vi "from string.vi"(8 "error in":errorcluster, 9 "data":string, 10 "version":string, 11 "Daqmx Module configuration in":refnum<class "Daqmx Module configuration.lvclass">) -> (0 "error out":errorcluster, 3 "Daqmx Module configuration out":refnum<class "Daqmx Module configuration.lvclass">)   [LabVIEW 2015, in "DAQmx Module Configuration.lvclass"]
doc: "Provides an interface for loading a module configuration from a file or other serialized data source. It is recommended that all children of this class store data in two sets--data required for its own initialization, and any data required for parent initialization--and that each implementation uses the <b>Call Parent Method</b> primitive to de-serialize parent information. As a result, it is expected that every module configuration class calls <b>component configuration.lvclass:From String.vi</b>."
uses:
  Daqmx Module configuration.lvclass
  Line.ctl
  <vilib>/NI/Tag Bus Module Framework/channel/TBM channel.lvclass
  Measurement Type.ctl
  Parameters.ctl
  Daqmx Module Configuration 1_0_0 Typedef.ctl
  Daqmx Module configuration.lvclass/Daqmx Module configuration.ctl
  <vilib>/NI/Tag Bus Module Framework/module configuration/TBM module configuration.lvclass
  <vilib>/NI/Configuration Framework/serializable configuration/NISE_CEF_serializable configuration.lvclass
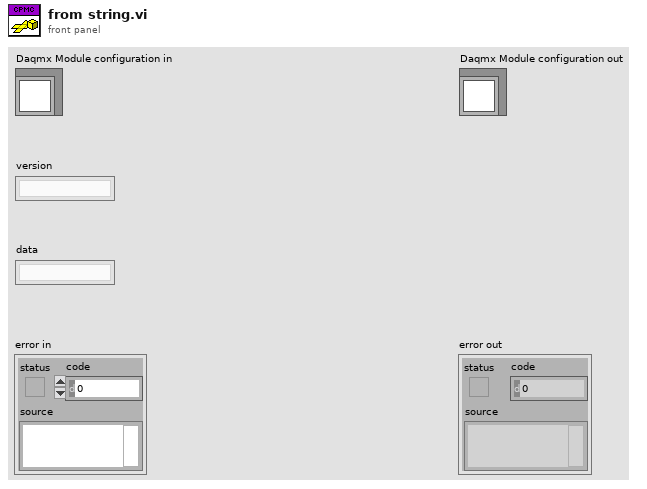
[diagram p1: front panel]
types:
  T1 = typedef "Daqmx Module configuration.lvclass/Daqmx Module Configuration 1_0_0 Typedef.ctl" = cluster{"channel":refnum<class "TBM channel.lvclass">, "Physical Channel":string, "Measurement Type":T2, "Parameters":cluster{"Digital Config":cluster{"Invert Lines?":bool}, "Voltage Config":cluster{"Maximum Value (V)":dbl, "Minimum Value (V)":dbl, "in terminal configuration (V)":i32, "out terminal configuration (V)":i32}, "Current Config":cluster{"Maximum Value (A)":dbl, "Minimum Value (A)":dbl, "shunt resistor location":i32, "input terminal configuration (C)":i32, "external shunt resistor value":dbl}, "RTD Config":cluster{"Maximum Value (°C)":dbl, "Minimum Value (°C)":dbl, "resistance configuration":i32, "r0":dbl, "current excitation value":dbl, "rtd type":i32, "current excitation source":i32}, "Thermocouple Config":cluster{"Minimum Value (C)":dbl, "Maximum Value (C)":dbl, "thermocouple type":i32, "cjc source":i32, "cjc value":dbl}, "Strain Config":cluster{"Maximum Value":dbl, "Minimum Value":dbl, "bridge information":cluster{"strain configuration":i32, "lead wire resistance":dbl, "initial bridge voltage":dbl, "voltage excitation source":i32, "voltage excitation value":dbl}, "strain gage information":cluster{"gage factor":dbl, "nominal gage resistance":dbl, "poisson ratio":dbl}}}}
  T2 = typedef "DAQmx Module Configuration.lvclass/Measurement Type.ctl" = enum16{"Digital Input", "Digital Output", "Voltage Input", "Voltage Output", "Current Input", "Current Output", "RTD", "Thermocouple", "Strain", "PWM"}
  T3 = typedef "DAQmx Module Configuration.lvclass/Line.ctl" = cluster{"Channel Array":refnum<class "TBM channel.lvclass">[], "Physical Channel":string, "Measurement Type":T2, "Parameters":T4}
  T4 = typedef "DAQmx Module Configuration.lvclass/Parameters.ctl" = cluster{"Digital Config":cluster{"Invert Lines?":bool}, "Voltage Config":cluster{"Maximum Value (V)":dbl, "Minimum Value (V)":dbl, "in terminal configuration (V)":i32, "out terminal configuration (V)":i32}, "Current Config":cluster{"Maximum Value (A)":dbl, "Minimum Value (A)":dbl, "shunt resistor location":i32, "input terminal configuration (C)":i32, "external shunt resistor value":dbl}, "RTD Config":cluster{"Maximum Value (°C)":dbl, "Minimum Value (°C)":dbl, "resistance configuration":i32, "r0":dbl, "current excitation value":dbl, "rtd type":i32, "current excitation source":i32}, "Thermocouple Config":cluster{"Minimum Value (C)":dbl, "Maximum Value (C)":dbl, "thermocouple type":i32, "cjc source":i32, "cjc value":dbl}, "Strain Config":cluster{"Maximum Value":dbl, "Minimum Value":dbl, "bridge information":cluster{"strain configuration":i32, "lead wire resistance":dbl, "initial bridge voltage":dbl, "voltage excitation source":i32, "voltage excitation value":dbl}, "strain gage information":cluster{"gage factor":dbl, "nominal gage resistance":dbl, "poisson ratio":dbl}}, "PWM Config":cluster{"Idle State":bool}}
  T5 = cluster{"Digital Config":cluster{"Invert Lines?":bool}, "Voltage Config":cluster{"Maximum Value (V)":dbl, "Minimum Value (V)":dbl, "in terminal configuration (V)":i32, "out terminal configuration (V)":i32}, "Current Config":cluster{"Maximum Value (A)":dbl, "Minimum Value (A)":dbl, "shunt resistor location":i32, "input terminal configuration (C)":i32, "external shunt resistor value":dbl}, "RTD Config":cluster{"Maximum Value (°C)":dbl, "Minimum Value (°C)":dbl, "resistance configuration":i32, "r0":dbl, "current excitation value":dbl, "rtd type":i32, "current excitation source":i32}, "Thermocouple Config":cluster{"Minimum Value (C)":dbl, "Maximum Value (C)":dbl, "thermocouple type":i32, "cjc source":i32, "cjc value":dbl}, "Strain Config":cluster{"Maximum Value":dbl, "Minimum Value":dbl, "bridge information":cluster{"strain configuration":i32, "lead wire resistance":dbl, "initial bridge voltage":dbl, "voltage excitation source":i32, "voltage excitation value":dbl}, "strain gage information":cluster{"gage factor":dbl, "nominal gage resistance":dbl, "poisson ratio":dbl}}}
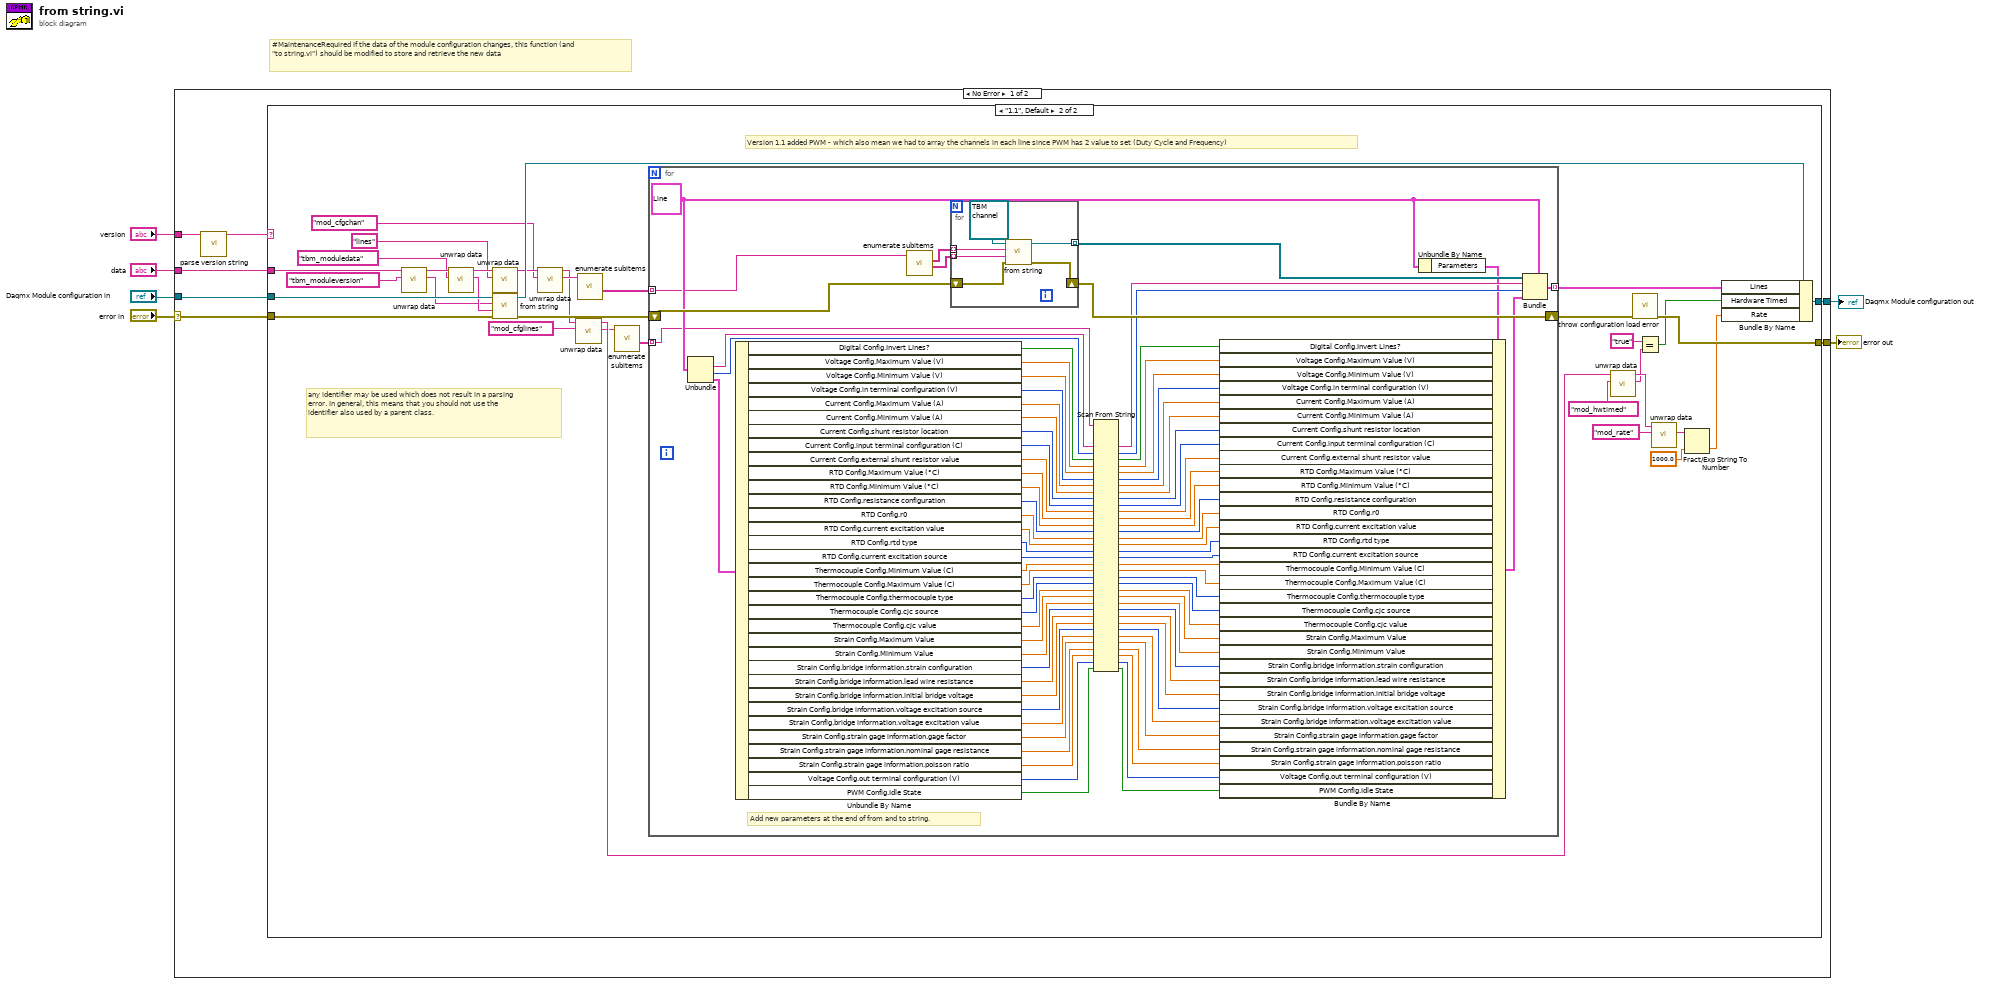
[diagram p0: block diagram]
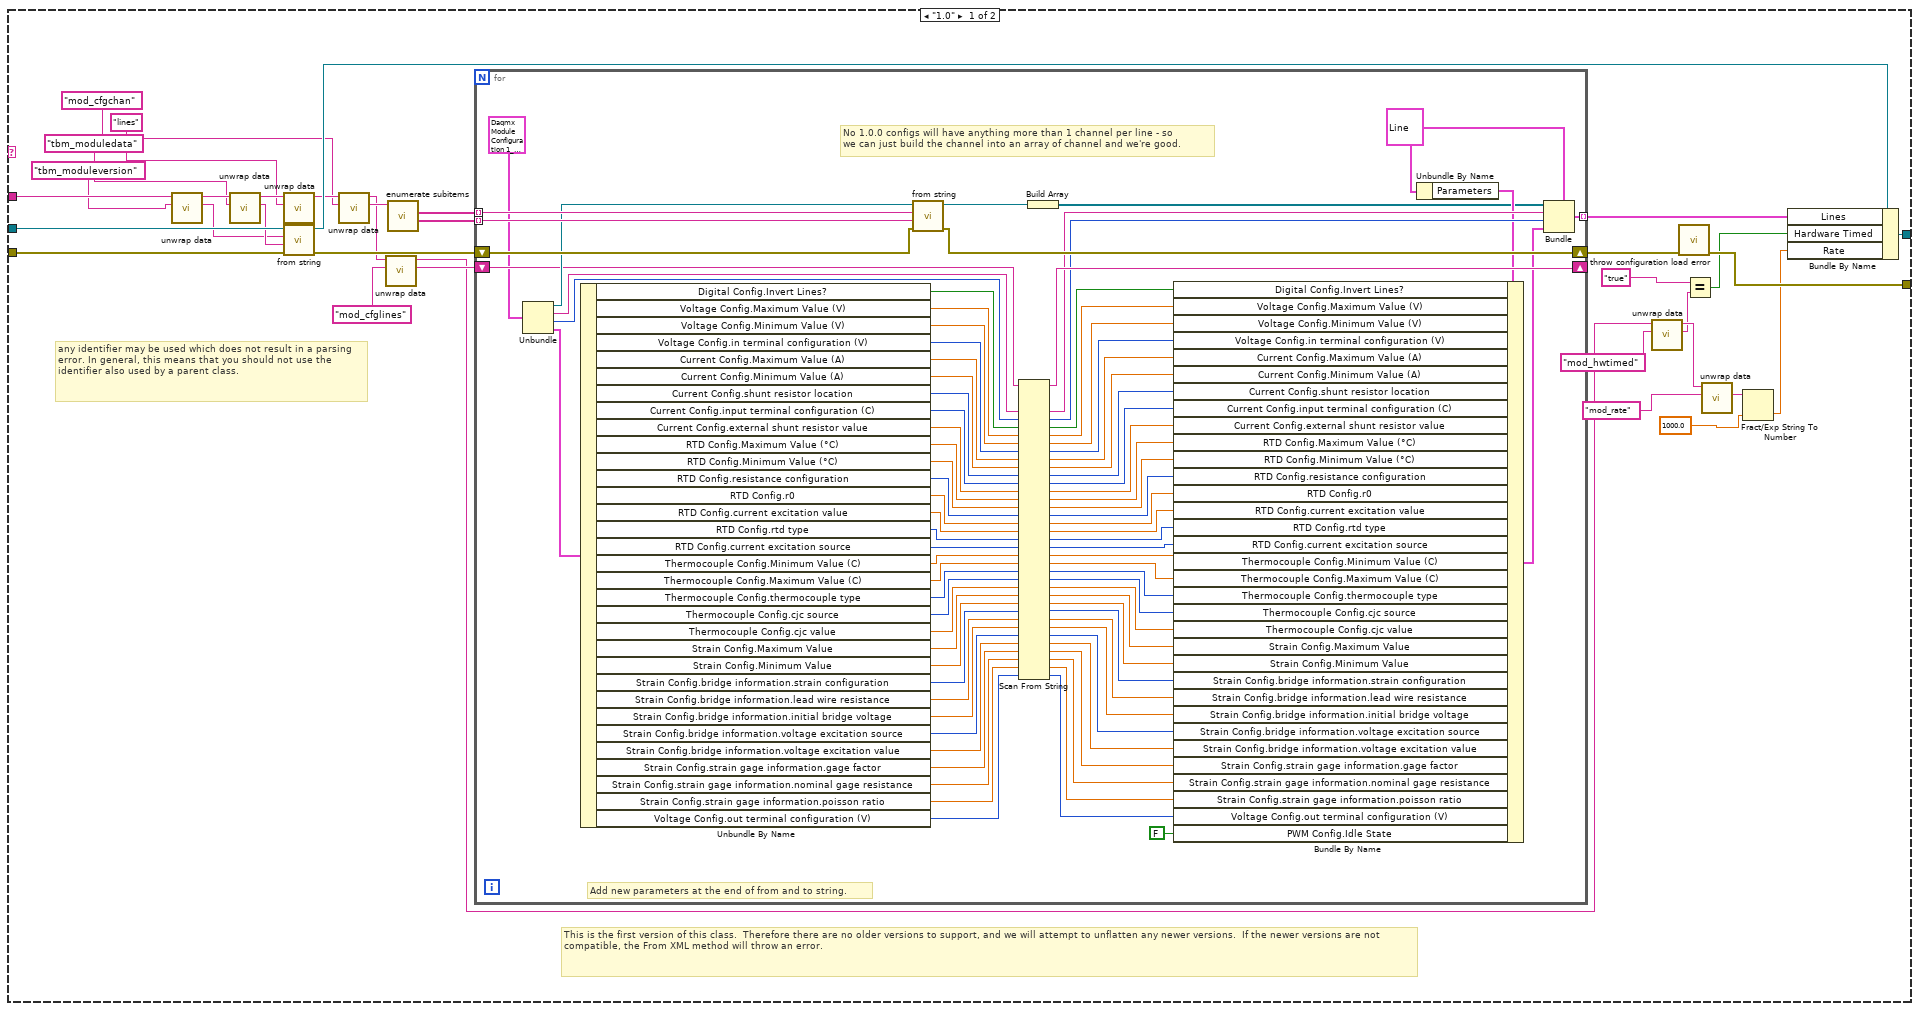
[diagram p2: hidden frame]
diagram:
  # "#MaintenanceRequired If the data of the module configuration changes, this function (and \"to string.vi\") should be modified to store and retrieve the new data"
  n1 = case shown="No Error" "error in" {
    selector: "error in" -> [w7 w255]
    tunnel: "data" -> [w13 _]
    tunnel: "Daqmx Module configuration in" -> [w12 w254]
    tunnel: [w11 w254] -> w1
    tunnel: [w10 w255] -> w6
    tunnel: "version" -> [w9 _]
    frame No Error {
      n2 = call <vilib>:"parse version string.vi"("full version"=w9) -> ("major.minor version"=w8:string)  [unwired: 7 in, 3 out]
      n3 = case shown="\"1.1\", Default" w8 {
        tunnel: w13 -> [w44 w162]
        tunnel: w7 -> [w43 w161]
        tunnel: w12 -> [w47 w165]
        tunnel: [w35 w153] -> w11
        tunnel: [w46 w164] -> w10
        frame "1.0" {
          # "This is the first version of this class.  Therefore there are no older versions to support, and we will attempt to unflatten any newer versions.  If the newer versions are not compatible, the From XML method will throw an error."
          # "any identifier may be used which does not result in a parsing error. In general, this means that you should not use the identifier also used by a parent class."
          n4 = call <vilib>:"unwrap data.vi"("identifier"="tbm_moduleversion" ("additional identifier"), "data to unwrap"=w44) -> ("unwrapped data"=w39:string, "remaining string"=w45:string)  [unwired: 8 in]
          n5 = call <vilib>:"unwrap data.vi"("identifier"="tbm_moduledata" ("additional identifier"), "data to unwrap"=w45) -> ("unwrapped data"=w41:string, "remaining string"=w38:string)  [unwired: 8 in]
          n6 = call <vilib>:"unwrap data.vi"("identifier"="lines" ("additional identifier"), "data to unwrap"=w38) -> ("remaining string"=w34:string)  [unwired: 8 in, 1 out]
          n7 = call-parent "from string.vi"("error in"=w43, "data"=w41, "version"=w39, "module configuration in"=w47) -> ("error out"=w30:errorcluster, "module configuration out"=w36:refnum<class "Daqmx Module configuration.lvclass">)  [unwired: 6 in]
          n8 = call <vilib>:"unwrap data.vi"("identifier"="mod_cfgchan", "data to unwrap"=w34) -> ("unwrapped data"=w29:string, "remaining string"=w26:string)  [unwired: 8 in]
          n9 = call <vilib>:"unwrap data.vi"("identifier"="mod_cfglines", "data to unwrap"=w26) -> ("unwrapped data"=w24:string, "remaining string"=w14:string)  [unwired: 8 in]
          n10 = call <vilib>:"enumerate subitems.vi"("data to enumerate"=w29) -> ("associated data"=w31:string[], "discovered subitems"=w32:string[])  [unwired: 8 in, 1 out]
          n11 = for {
            shift-right: [w126] -> w28
            shift-left: w30 -> [w131]
            tunnel: w32 -> [w130] mode=indexing
            tunnel: w31 -> [w129] mode=indexing
            tunnel: [w127] -> w27 mode=indexing
            shift-right: [w98] -> _
            shift-left: w24 -> [w99]
            w54 = T3 {"Channel Array"=[], "Physical Channel"="", "Measurement Type"=enum."Digital Input", "Parameters"={"Digital Config"={"Invert Lines?"=FALSE}, "Voltage Config"={"Maximum Value (V)"=5.0, "Minimum Value (V)"=-5.0, "in terminal configuration (V)"=-1, "out terminal configuration (V)"=-1}, "Current Config"={"Maximum Value (A)"=0.02, "Minimum Value (A)"=0.0, "shunt resistor location"=-1, "input terminal configuration (C)"=-1, "external shunt resistor value"=249.0}, "RTD Config"={"Maximum Value (°C)"=100.0, "Minimum Value (°C)"=0.0, "resistance configuration"=2, "r0"=100.0, "current excitation value"=0.0025, "rtd type"=10137, "current excitation source"=10167}, "Thermocouple Config"={"Minimum Value (C)"=0.0, "Maximum Value (C)"=100.0, "thermocouple type"=10072, "cjc source"=10116, "cjc value"=25.0}, "Strain Config"={"Maximum Value"=0.001, "Minimum Value"=-0.001, "bridge information"={"strain configuration"=10183, "lead wire resistance"=0.0, "initial bridge voltage"=0.0, "voltage excitation source"=10200, "voltage excitation value"=2.5}, "strain gage information"={"gage factor"=2.0, "nominal gage resistance"=350.0, "poisson ratio"=0.3}}, "PWM Config"={"Idle State"=FALSE}}} ("Line")
            # "No 1.0.0 configs will have anything more than 1 channel per line - so\nwe can just build the channel into an array of channel and we're good."
            # "Add new parameters at the end of from and to string."
            n12 = Unbundle(T1 {"channel"=refnum, "Physical Channel"="", "Measurement Type"=enum."Digital Input", "Parameters"={"Digital Config"={"Invert Lines?"=FALSE}, "Voltage Config"={"Maximum Value (V)"=5.0, "Minimum Value (V)"=-5.0, "in terminal configuration (V)"=-1, "out terminal configuration (V)"=-1}, "Current Config"={"Maximum Value (A)"=0.02, "Minimum Value (A)"=0.0, "shunt resistor location"=-1, "input terminal configuration (C)"=-1, "external shunt resistor value"=249.0}, "RTD Config"={"Maximum Value (°C)"=100.0, "Minimum Value (°C)"=0.0, "resistance configuration"=2, "r0"=100.0, "current excitation value"=0.0025, "rtd type"=10137, "current excitation source"=10167}, "Thermocouple Config"={"Minimum Value (C)"=0.0, "Maximum Value (C)"=100.0, "thermocouple type"=10072, "cjc source"=10116, "cjc value"=25.0}, "Strain Config"={"Maximum Value"=0.001, "Minimum Value"=-0.001, "bridge information"={"strain configuration"=10183, "lead wire resistance"=0.0, "initial bridge voltage"=0.0, "voltage excitation source"=10200, "voltage excitation value"=2.5}, "strain gage information"={"gage factor"=2.0, "nominal gage resistance"=350.0, "poisson ratio"=0.3}}}} ("1.0 Config")) -> ("channel"=w125:refnum<class "TBM channel.lvclass">, "Physical Channel"=w124:string, "Measurement Type"=w100:T2, "Parameters"=w96:T5)
            n13 = Unbundle By Name(w96) -> ("Digital Config.Invert Lines?"=w123:bool, "Voltage Config.Maximum Value (V)"=w122:dbl, "Voltage Config.Minimum Value (V)"=w121:dbl, "Voltage Config.in terminal configuration (V)"=w120:i32, "Current Config.Maximum Value (A)"=w119:dbl, "Current Config.Minimum Value (A)"=w118:dbl, "Current Config.shunt resistor location"=w117:i32, "Current Config.input terminal configuration (C)"=w116:i32, "Current Config.external shunt resistor value"=w114:dbl, "RTD Config.Maximum Value (°C)"=w115:dbl, "RTD Config.Minimum Value (°C)"=w113:dbl, "RTD Config.resistance configuration"=w112:i32, "RTD Config.r0"=w111:dbl, "RTD Config.current excitation value"=w110:dbl, "RTD Config.rtd type"=w109:i32, "RTD Config.current excitation source"=w108:i32, "Thermocouple Config.Minimum Value (C)"=w107:dbl, "Thermocouple Config.Maximum Value (C)"=w106:dbl, "Thermocouple Config.thermocouple type"=w105:i32, "Thermocouple Config.cjc source"=w104:i32, "Thermocouple Config.cjc value"=w103:dbl, "Strain Config.Maximum Value"=w102:dbl, "Strain Config.Minimum Value"=w101:dbl, "Strain Config.bridge information.strain configuration"=w95:i32, "Strain Config.bridge information.lead wire resistance"=w94:dbl, "Strain Config.bridge information.initial bridge voltage"=w93:dbl, "Strain Config.bridge information.voltage excitation source"=w92:i32, "Strain Config.bridge information.voltage excitation value"=w91:dbl, "Strain Config.strain gage information.gage factor"=w90:dbl, "Strain Config.strain gage information.nominal gage resistance"=w89:dbl, "Strain Config.strain gage information.poisson ratio"=w88:dbl, "Voltage Config.out terminal configuration (V)"=w52:i32)
            n14 = call-dynamic "from string.vi"("error in"=w131, "channel data"=w129, "identifier"=w130, "channel in"=w125) -> ("error out"=w126:errorcluster, "channel out"=w128:refnum<class "TBM channel.lvclass">)  [unwired: 6 in]
            n15 = Scan From String(input string=w99, default 1=w124, default 2=w100, default 3=w123, default 4=w122, default 5=w121, default 6=w120, default 7=w119, default 8=w118, default 9=w117, default 10=w116, default 11=w114, default 12=w115, default 13=w113, default 14=w112, default 15=w111, default 16=w110, default 17=w109, default 18=w108, default 19=w107, default 20=w106, default 21=w105, default 22=w104, default 23=w103, default 24=w102, default 25=w101, default 26=w95, default 27=w94, default 28=w93, default 29=w92, default 30=w91, default 31=w90, default 32=w89, default 33=w88, default 34=w52) -> (remaining string=w98:string, output 1=w97:string, output 2=w87:T2, output 3=w86:bool, output 4=w85:dbl, output 5=w84:dbl, output 6=w83:i32, output 7=w82:dbl, output 8=w81:dbl, output 9=w80:i32, output 10=w79:i32, output 11=w78:dbl, output 12=w77:dbl, output 13=w76:dbl, output 14=w75:i32, output 15=w74:dbl, output 16=w73:dbl, output 17=w72:i32, output 18=w71:i32, output 19=w70:dbl, output 20=w69:dbl, output 21=w68:i32, output 22=w67:i32, output 23=w66:dbl, output 24=w65:dbl, output 25=w64:dbl, output 26=w63:i32, output 27=w62:dbl, output 28=w61:dbl, output 29=w60:i32, output 30=w59:dbl, output 31=w58:dbl, output 32=w57:dbl, output 33=w56:dbl, output 34=w51:i32)  [unwired: 3 in, 2 out]
            n16 = Build Array(w128) -> (w50:refnum<class "TBM channel.lvclass">[])
            n17 = Unbundle By Name(w54) -> ("Parameters"=w53:T4)
            n18 = Bundle By Name(cluster=w53, "Digital Config.Invert Lines?"=w86, "Voltage Config.Maximum Value (V)"=w85, "Voltage Config.Minimum Value (V)"=w84, "Voltage Config.in terminal configuration (V)"=w83, "Current Config.Maximum Value (A)"=w82, "Current Config.Minimum Value (A)"=w81, "Current Config.shunt resistor location"=w80, "Current Config.input terminal configuration (C)"=w79, "Current Config.external shunt resistor value"=w78, "RTD Config.Maximum Value (°C)"=w77, "RTD Config.Minimum Value (°C)"=w76, "RTD Config.resistance configuration"=w75, "RTD Config.r0"=w74, "RTD Config.current excitation value"=w73, "RTD Config.rtd type"=w72, "RTD Config.current excitation source"=w71, "Thermocouple Config.Minimum Value (C)"=w70, "Thermocouple Config.Maximum Value (C)"=w69, "Thermocouple Config.thermocouple type"=w68, "Thermocouple Config.cjc source"=w67, "Thermocouple Config.cjc value"=w66, "Strain Config.Maximum Value"=w65, "Strain Config.Minimum Value"=w64, "Strain Config.bridge information.strain configuration"=w63, "Strain Config.bridge information.lead wire resistance"=w62, "Strain Config.bridge information.initial bridge voltage"=w61, "Strain Config.bridge information.voltage excitation source"=w60, "Strain Config.bridge information.voltage excitation value"=w59, "Strain Config.strain gage information.gage factor"=w58, "Strain Config.strain gage information.nominal gage resistance"=w57, "Strain Config.strain gage information.poisson ratio"=w56, "Voltage Config.out terminal configuration (V)"=w51, "PWM Config.Idle State"=FALSE) -> (w55:T4)
            n19 = Bundle(cluster=w54, "Channel Array"=w50, "Physical Channel"=w97, "Measurement Type"=w87, "Parameters"=w55) -> (w127:T3)
          }
          n20 = call <vilib>:"unwrap data.vi"("identifier"="mod_hwtimed", "data to unwrap"=w14) -> ("unwrapped data"=w20:string, "remaining string"=w21:string)  [unwired: 8 in]
          n21 = call <vilib>:"throw configuration load error.vi"("error in"=w28) -> ("error out"=w46:errorcluster)  [unwired: 10 in]
          n22 = Equal?(x="true" ("identifier"), y=w20) -> (x = y?=w18:bool)
          n23 = call <vilib>:"unwrap data.vi"("identifier"="mod_rate", "data to unwrap"=w21) -> ("unwrapped data"=w17:string)  [unwired: 8 in, 1 out]
          n24 = Fract/Exp String To Number(string=w17, default (0 dbl)=1000.0 ("default (0 DBL)")) -> (number=w16:dbl)  [unwired: 2 in, 1 out]
          n25 = Bundle By Name(cluster=w36, "Lines"=w27, "Hardware Timed"=w18, "Rate"=w16) -> (w35:refnum<class "Daqmx Module configuration.lvclass">)
        }
        frame "1.1", Default {
          # "Version 1.1 added PWM - which also mean we had to array the channels in each line since PWM has 2 value to set (Duty Cycle and Frequency)"
          # "any identifier may be used which does not result in a parsing error. In general, this means that you should not use the identifier also used by a parent class."
          n26 = call <vilib>:"unwrap data.vi"("identifier"="tbm_moduleversion" ("additional identifier"), "data to unwrap"=w162) -> ("unwrapped data"=w157:string, "remaining string"=w163:string)  [unwired: 8 in]
          n27 = call <vilib>:"unwrap data.vi"("identifier"="tbm_moduledata" ("additional identifier"), "data to unwrap"=w163) -> ("unwrapped data"=w159:string, "remaining string"=w156:string)  [unwired: 8 in]
          n28 = call <vilib>:"unwrap data.vi"("identifier"="lines" ("additional identifier"), "data to unwrap"=w156) -> ("remaining string"=w152:string)  [unwired: 8 in, 1 out]
          n29 = call-parent "from string.vi"("error in"=w161, "data"=w159, "version"=w157, "module configuration in"=w165) -> ("error out"=w149:errorcluster, "module configuration out"=w154:refnum<class "Daqmx Module configuration.lvclass">)  [unwired: 6 in]
          n30 = call <vilib>:"unwrap data.vi"("identifier"="mod_cfgchan", "data to unwrap"=w152) -> ("unwrapped data"=w148:string, "remaining string"=w145:string)  [unwired: 8 in]
          n31 = call <vilib>:"unwrap data.vi"("identifier"="mod_cfglines", "data to unwrap"=w145) -> ("unwrapped data"=w133:string, "remaining string"=w134:string)  [unwired: 8 in]
          n32 = call <vilib>:"enumerate subitems.vi"("data to enumerate"=w148) -> ("associated data"=w150:string[])  [unwired: 8 in, 2 out]
          n33 = call <vilib>:"enumerate subitems.vi"("data to enumerate"=w133) -> ("associated data"=w132:string[])  [unwired: 8 in, 2 out]
          n34 = for {
            shift-right: [w244] -> w147
            shift-left: w149 -> [w247]
            tunnel: w150 -> [w167] mode=indexing
            tunnel: [w245] -> w146 mode=indexing
            tunnel: w132 -> [w166] mode=indexing
            w175 = T3 {"Channel Array"=[], "Physical Channel"="", "Measurement Type"=enum."Digital Input", "Parameters"={"Digital Config"={"Invert Lines?"=FALSE}, "Voltage Config"={"Maximum Value (V)"=5.0, "Minimum Value (V)"=-5.0, "in terminal configuration (V)"=-1, "out terminal configuration (V)"=-1}, "Current Config"={"Maximum Value (A)"=0.02, "Minimum Value (A)"=0.0, "shunt resistor location"=-1, "input terminal configuration (C)"=-1, "external shunt resistor value"=249.0}, "RTD Config"={"Maximum Value (°C)"=100.0, "Minimum Value (°C)"=0.0, "resistance configuration"=2, "r0"=100.0, "current excitation value"=0.0025, "rtd type"=10137, "current excitation source"=10167}, "Thermocouple Config"={"Minimum Value (C)"=0.0, "Maximum Value (C)"=100.0, "thermocouple type"=10072, "cjc source"=10116, "cjc value"=25.0}, "Strain Config"={"Maximum Value"=0.001, "Minimum Value"=-0.001, "bridge information"={"strain configuration"=10183, "lead wire resistance"=0.0, "initial bridge voltage"=0.0, "voltage excitation source"=10200, "voltage excitation value"=2.5}, "strain gage information"={"gage factor"=2.0, "nominal gage resistance"=350.0, "poisson ratio"=0.3}}, "PWM Config"={"Idle State"=FALSE}}} ("Line")
            # "Add new parameters at the end of from and to string."
            n35 = Unbundle(w175) -> ("Physical Channel"=w243:string, "Measurement Type"=w219:T2, "Parameters"=w217:T4)  [unwired: 1 out]
            n36 = Unbundle By Name(w217) -> ("Digital Config.Invert Lines?"=w242:bool, "Voltage Config.Maximum Value (V)"=w241:dbl, "Voltage Config.Minimum Value (V)"=w240:dbl, "Voltage Config.in terminal configuration (V)"=w239:i32, "Current Config.Maximum Value (A)"=w238:dbl, "Current Config.Minimum Value (A)"=w237:dbl, "Current Config.shunt resistor location"=w236:i32, "Current Config.input terminal configuration (C)"=w235:i32, "Current Config.external shunt resistor value"=w233:dbl, "RTD Config.Maximum Value (°C)"=w234:dbl, "RTD Config.Minimum Value (°C)"=w232:dbl, "RTD Config.resistance configuration"=w231:i32, "RTD Config.r0"=w230:dbl, "RTD Config.current excitation value"=w229:dbl, "RTD Config.rtd type"=w228:i32, "RTD Config.current excitation source"=w227:i32, "Thermocouple Config.Minimum Value (C)"=w226:dbl, "Thermocouple Config.Maximum Value (C)"=w225:dbl, "Thermocouple Config.thermocouple type"=w224:i32, "Thermocouple Config.cjc source"=w223:i32, "Thermocouple Config.cjc value"=w222:dbl, "Strain Config.Maximum Value"=w221:dbl, "Strain Config.Minimum Value"=w220:dbl, "Strain Config.bridge information.strain configuration"=w216:i32, "Strain Config.bridge information.lead wire resistance"=w215:dbl, "Strain Config.bridge information.initial bridge voltage"=w214:dbl, "Strain Config.bridge information.voltage excitation source"=w213:i32, "Strain Config.bridge information.voltage excitation value"=w212:dbl, "Strain Config.strain gage information.gage factor"=w211:dbl, "Strain Config.strain gage information.nominal gage resistance"=w210:dbl, "Strain Config.strain gage information.poisson ratio"=w209:dbl, "Voltage Config.out terminal configuration (V)"=w173:i32, "PWM Config.Idle State"=w171:bool)
            n37 = call <vilib>:"enumerate subitems.vi"("data to enumerate"=w167) -> ("associated data"=w168:string[], "discovered subitems"=w169:string[])  [unwired: 8 in, 1 out]
            n38 = for {
              tunnel: w169 -> [w250] mode=indexing
              tunnel: w168 -> [w249] mode=indexing
              tunnel: [w252] -> w246 mode=indexing
              shift-right: [w251] -> w244
              shift-left: w247 -> [w253]
              n39 = call-dynamic "from string.vi"("error in"=w253, "channel data"=w249, "identifier"=w250, "channel in"=refnum<class "TBM channel.lvclass"> refnum) -> ("error out"=w251:errorcluster, "channel out"=w252:refnum<class "TBM channel.lvclass">)  [unwired: 6 in]
            }
            n40 = Scan From String(input string=w166, default 1=w243, default 2=w219, default 3=w242, default 4=w241, default 5=w240, default 6=w239, default 7=w238, default 8=w237, default 9=w236, default 10=w235, default 11=w233, default 12=w234, default 13=w232, default 14=w231, default 15=w230, default 16=w229, default 17=w228, default 18=w227, default 19=w226, default 20=w225, default 21=w224, default 22=w223, default 23=w222, default 24=w221, default 25=w220, default 26=w216, default 27=w215, default 28=w214, default 29=w213, default 30=w212, default 31=w211, default 32=w210, default 33=w209, default 34=w173, default 35=w171) -> (output 1=w218:string, output 2=w208:T2, output 3=w207:bool, output 4=w206:dbl, output 5=w205:dbl, output 6=w204:i32, output 7=w203:dbl, output 8=w202:dbl, output 9=w201:i32, output 10=w200:i32, output 11=w199:dbl, output 12=w198:dbl, output 13=w197:dbl, output 14=w196:i32, output 15=w195:dbl, output 16=w194:dbl, output 17=w193:i32, output 18=w192:i32, output 19=w191:dbl, output 20=w190:dbl, output 21=w189:i32, output 22=w188:i32, output 23=w187:dbl, output 24=w186:dbl, output 25=w185:dbl, output 26=w184:i32, output 27=w183:dbl, output 28=w182:dbl, output 29=w181:i32, output 30=w180:dbl, output 31=w179:dbl, output 32=w178:dbl, output 33=w177:dbl, output 34=w172:i32, output 35=w170:bool)  [unwired: 3 in, 3 out]
            n41 = Unbundle By Name(w175) -> ("Parameters"=w174:T4)
            n42 = Bundle By Name(cluster=w174, "Digital Config.Invert Lines?"=w207, "Voltage Config.Maximum Value (V)"=w206, "Voltage Config.Minimum Value (V)"=w205, "Voltage Config.in terminal configuration (V)"=w204, "Current Config.Maximum Value (A)"=w203, "Current Config.Minimum Value (A)"=w202, "Current Config.shunt resistor location"=w201, "Current Config.input terminal configuration (C)"=w200, "Current Config.external shunt resistor value"=w199, "RTD Config.Maximum Value (°C)"=w198, "RTD Config.Minimum Value (°C)"=w197, "RTD Config.resistance configuration"=w196, "RTD Config.r0"=w195, "RTD Config.current excitation value"=w194, "RTD Config.rtd type"=w193, "RTD Config.current excitation source"=w192, "Thermocouple Config.Minimum Value (C)"=w191, "Thermocouple Config.Maximum Value (C)"=w190, "Thermocouple Config.thermocouple type"=w189, "Thermocouple Config.cjc source"=w188, "Thermocouple Config.cjc value"=w187, "Strain Config.Maximum Value"=w186, "Strain Config.Minimum Value"=w185, "Strain Config.bridge information.strain configuration"=w184, "Strain Config.bridge information.lead wire resistance"=w183, "Strain Config.bridge information.initial bridge voltage"=w182, "Strain Config.bridge information.voltage excitation source"=w181, "Strain Config.bridge information.voltage excitation value"=w180, "Strain Config.strain gage information.gage factor"=w179, "Strain Config.strain gage information.nominal gage resistance"=w178, "Strain Config.strain gage information.poisson ratio"=w177, "Voltage Config.out terminal configuration (V)"=w172, "PWM Config.Idle State"=w170) -> (w176:T4)
            n43 = Bundle(cluster=w175, "Channel Array"=w246, "Physical Channel"=w218, "Measurement Type"=w208, "Parameters"=w176) -> (w245:T3)
          }
          n44 = call <vilib>:"unwrap data.vi"("identifier"="mod_hwtimed", "data to unwrap"=w134) -> ("unwrapped data"=w140:string, "remaining string"=w141:string)  [unwired: 8 in]
          n45 = call <vilib>:"throw configuration load error.vi"("error in"=w147) -> ("error out"=w164:errorcluster)  [unwired: 10 in]
          n46 = Equal?(x="true" ("identifier"), y=w140) -> (x = y?=w138:bool)
          n47 = call <vilib>:"unwrap data.vi"("identifier"="mod_rate", "data to unwrap"=w141) -> ("unwrapped data"=w137:string)  [unwired: 8 in, 1 out]
          n48 = Fract/Exp String To Number(string=w137, default (0 dbl)=1000.0 ("default (0 DBL)")) -> (number=w136:dbl)  [unwired: 2 in, 1 out]
          n49 = Bundle By Name(cluster=w154, "Lines"=w146, "Hardware Timed"=w138, "Rate"=w136) -> (w153:refnum<class "Daqmx Module configuration.lvclass">)
        }
      }
    }
    frame Error {
    }
  }
  "error out" <- w6
  "Daqmx Module configuration out" <- w1
